vi "SLSC_Example_AsyscRTEnginer.vi"(10 "Parameters":variant, 11 "Process":refnum<class "Process.lvclass">) -> ()   [LabVIEW 2020, in "SLSC EDS Engine.lvlib"]
uses:
  SLSC EDS Engine.lvlib
  <vilib>/NI/NIVS Inline Async API/_VS Inline Async API/Process/Process.lvclass
  Types/Async Engine State Control.ctl
  Shared/Compiled.Settings.ctl
  Shared/SLSC Static Settings.ctl
  SLSC CD API/SLSC CD Engine/SLSC Dynamic Channel.ctl
  SLSC CD API/SLSC CD Engine/SLSC Datatype.ctl
  <vilib>/NI/NIVS Inline Async API/_VS Inline Async API/Process/Process.lvclass/Process.ctl
  <vilib>/NI/NIVS Inline Async API/_Data Access Engine/Access Type Classes/Read/Read.lvclass/Read.ctl
  <vilib>/NI/NIVS Inline Async API/_Data Access Engine/Access Type Classes/ReadWrite/ReadWrite.lvclass/ReadWrite.ctl
  <vilib>/NI/NIVS Inline Async API/_Data Access Engine/Access Type Classes/Write/Write.lvclass/Write.ctl
  <vilib>/NI/NIVS Inline Async API/_Data Access Engine/Data Access Engine/Methods/Read.Data.Detect.vi
  <vilib>/NI/NIVS Inline Async API/_Data Access Engine/Data Access Engine/Methods/Write.Data.vi
  <vilib>/NI/NIVS Inline Async API/_Data Access Engine/Data Access Engine/Methods/ReadWrite.Data.vi
  <vilib>/NI/NIVS Inline Async API/_VS Inline Async API/Process/Data Member Access/Read Data Access.vi
  <vilib>/NI/NIVS Inline Async API/_VS Inline Async API/Error Handling Process/SubVIs/Error.ConvertArray.vi
  <vilib>/NI/NIVS Inline Async API/_Data Access Engine/Access Type Classes/Read/Read.ProcessData.Detect.vi
  <vilib>/NI/NIVS Inline Async API/_Data Access Engine/Access Type Classes/Write/Write.ProcessData.vi
  SLSC CD API/SLSC CD Shared/SLSC Define Resource Name.vi
  <vilib>/NI/NIVS Inline Async API/_Data Access Engine/Access Type Classes/ReadWrite/ReadWrite.ProcessData.vi
  <vilib>/NI/NIVS Inline Async API/_Data Access Engine/Access Type Classes/Write/Write.Buffer.vi
  <vilib>/NI/NIVS Inline Async API/_Data Access Engine/Access Type Classes/Write/Write.Commit.vi
  Shared/Constants.vi
  <vilib>/SLSC/Initialize Session with Devices.vi
  <vilib>/SLSC/Set Generic Property.vi
  <vilib>/SLSC/Set Generic Property (Bool).vi
  <vilib>/SLSC/Set Generic Property (DBL).vi
  <vilib>/SLSC/Set Generic Property (I32).vi
  <vilib>/SLSC/Set Generic Property (I64).vi
  <vilib>/SLSC/Set Generic Property (String).vi
  <vilib>/SLSC/Set Generic Property (U32).vi
  <vilib>/SLSC/Set Generic Property (U64).vi
  SLSC CD API/SLSC CD Shared/SLSC Error Suppression.vi
  <vilib>/SLSC/Commit Properties.vi
  <vilib>/SLSC/Commit Properties for Devices.vi
  <vilib>/SLSC/Execute Command.vi
  <vilib>/SLSC/Execute Device Command.vi
  <vilib>/SLSC/Execute Phys Chan Command.vi
  <vilib>/SLSC/Get Generic Property.vi
  <vilib>/SLSC/Get Generic Property (Bool).vi
  <vilib>/SLSC/Get Generic Property (DBL).vi
  <vilib>/SLSC/Get Generic Property (I32).vi
  <vilib>/SLSC/Get Generic Property (I64).vi
  <vilib>/SLSC/Get Generic Property (String).vi
  <vilib>/SLSC/Get Generic Property (U32).vi
  <vilib>/SLSC/Get Generic Property (U64).vi
  <vilib>/SLSC/Close Session.vi
  <vilib>/NI/NIVS Inline Async API/_Data Access Engine/Data Access Engine/Data Access Engine.lvclass
  <vilib>/NI/NIVS Inline Async API/_Data Access Engine/Data Access Engine/Methods/ReadWrite.Lookup.vi
  <vilib>/NI/NIVS Inline Async API/_Data Access Engine/Data Access Engine/Methods/Write.Lookup.vi
  <vilib>/NI/NIVS Inline Async API/_Data Access Engine/Data Access Engine/Methods/Read.Lookup.vi
  <vilib>/SLSC/SLSC.lvlib
  Shared/SLSC EDS Shared.lvlib
  SLSC CD API/SLSC CD Shared/SLSC CD Shared.lvlib
  SLSC CD API/SLSC CD Engine/SLSC CD Engine.lvlib
  <vilib>/NI VeriStand/Custom Device Tools/Custom Device Utility Library/Custom Device Utility Library.lvlib
  <vilib>/NI/NIVS Inline Async API/_Data Access Engine/Access Type Classes/Write/Write.lvclass
panel:
  out "LoopRate(ms)":u32=50
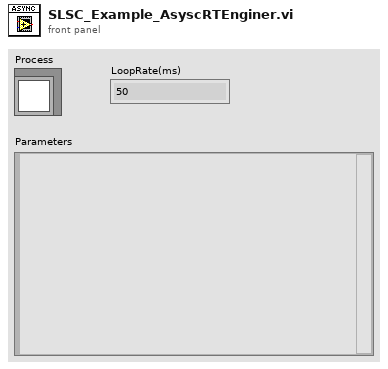
[diagram p1: front panel]
types:
  T1 = typedef "SLSC EDS Engine.lvlib/Async Engine State Control.ctl" = enum16{"Initialize", "Configure", "Run", "Reset", "Shutdown"}
  T2 = typedef "SLSC EDS Shared.lvlib/Compiled.Settings.ctl" = cluster{"Name":string, "SLSC Name or IP Address":string, "Slot #":i32, "Reservation Access":i32, "Reservation Group":string, "Configuration Data":T3, "SLSC Get/Read Properties":T4[], "SLSC Set/Write Properties":T4[], "SLSC Dynamic Commands":T4[], "Support Modules":cluster{"Dev.ProductNumber":u32, "Dev.VendorNumber":u32}[]}
  T3 = typedef "SLSC EDS Shared.lvlib/SLSC Static Settings.ctl" = cluster{"Properties":cluster{"Boolean Properties":cluster{"property":refnum<k21>, "Value":bool, "SLSC Item":refnum<k21>, "reset value":bool}[], "Double Properties":cluster{"property":refnum<k21>, "Double Write":dbl, "SLSC Item":refnum<k21>, "Double Reset Value":dbl}[], "I32 Properties":cluster{"property":refnum<k21>, "Int32 Write":i32, "SLSC Item":refnum<k21>, "Int32 Reset Value":i32}[], "I64 Properties":cluster{"property":refnum<k21>, "Int64 Write":i64, "SLSC Item":refnum<k21>, "Int64 Reset Value":i64}[], "String Properties":cluster{"property":refnum<k21>, "String Write":string, "SLSC Item":refnum<k21>, "String Reset Value":string}[], "U32 Properties":cluster{"property":refnum<k21>, "UInt32 Write":u32, "SLSC Item":refnum<k21>, "UInt32 Reset Value":u32}[], "U64 Properties":cluster{"property":refnum<k21>, "UInt64 Write":u64, "SLSC Item":refnum<k21>, "UInt64 Reset Value":u64}[]}, "Commands":T4[], "Reset Commands":T4[], "Apply Values on Deployment":bool, "Apply Reset on Undeployment":bool, "Change Commands":T4[]}
  T4 = typedef "SLSC CD Shared.lvlib/SLSC Dynamic Channel.ctl" = cluster{"SLSC Item":string, "property":string, "Data Type":T5}
  T5 = typedef "SLSC CD Shared.lvlib/SLSC Datatype.ctl" = enum16{"Bool", "Double", "I32", "I64", "String", "U32", "U64"}
  T6 = typedef "Data Access Engine.lvlib/Data Access Engine.lvclass/Write.DVR.ctl" = refnum<data-value>
  T7 = typedef "Data Access Engine.lvlib/Data Access Engine.lvclass/Read.DVR.ctl" = refnum<data-value>
  T8 = typedef "Data Access Engine.lvlib/Data Access Engine.lvclass/ReadWrite.DVR.ctl" = refnum<data-value>
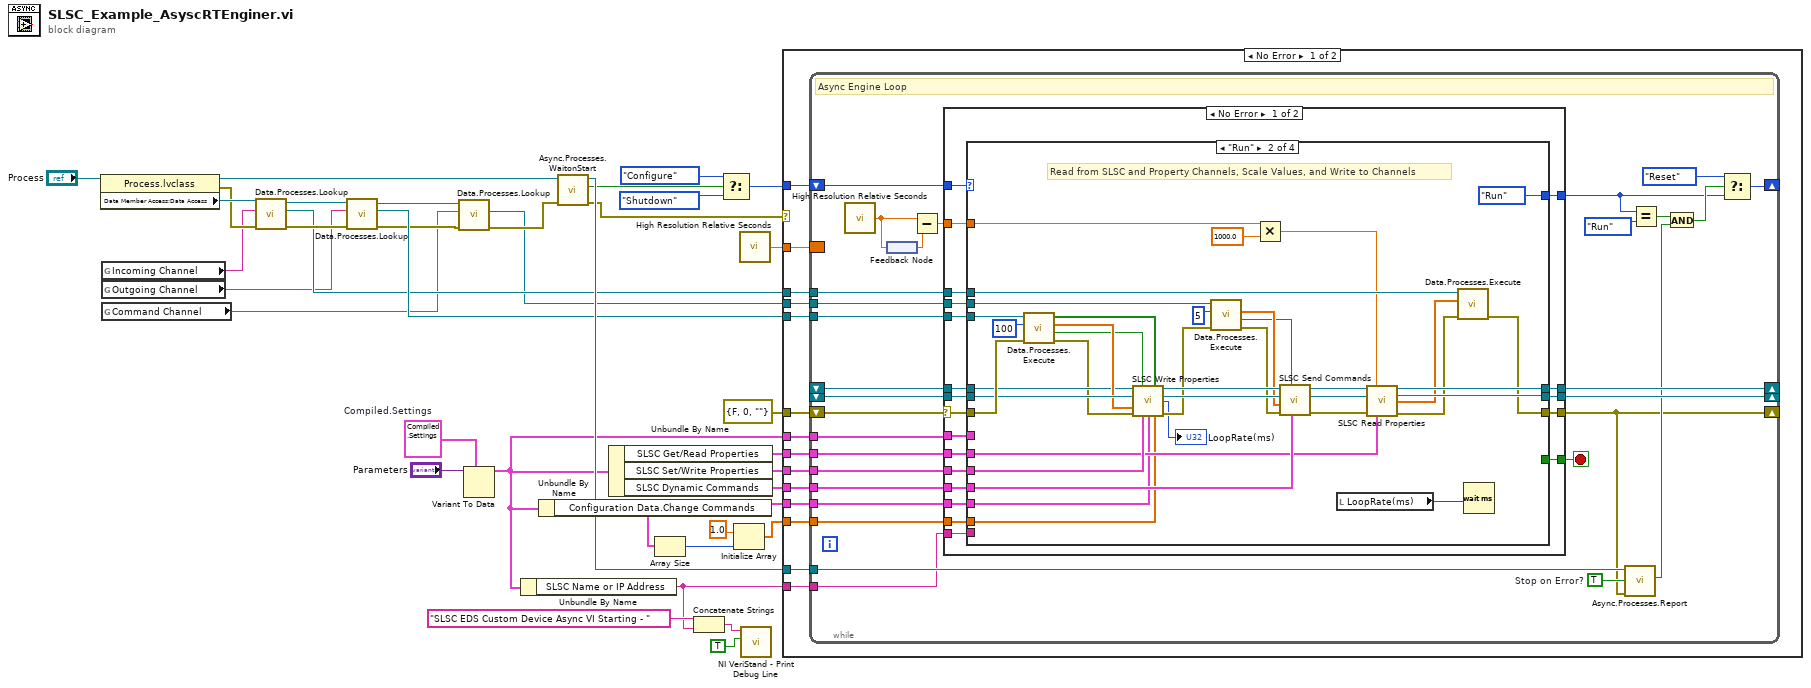
[diagram p0: block diagram]
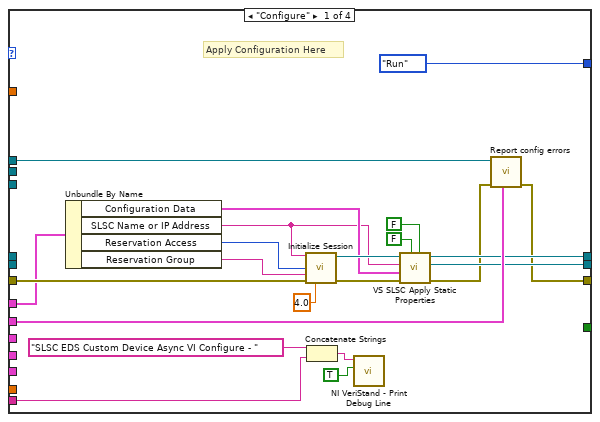
[diagram p2: hidden frame]
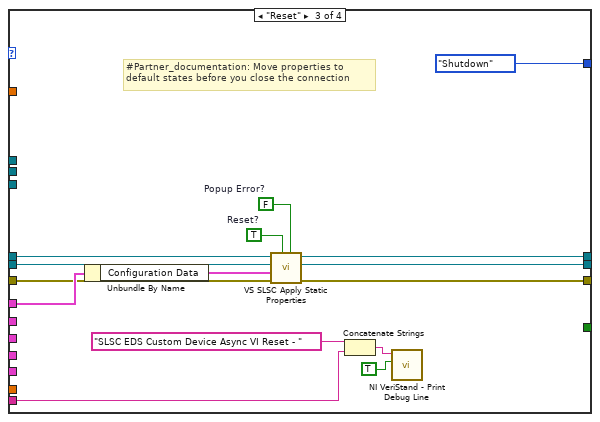
[diagram p3: hidden frame]
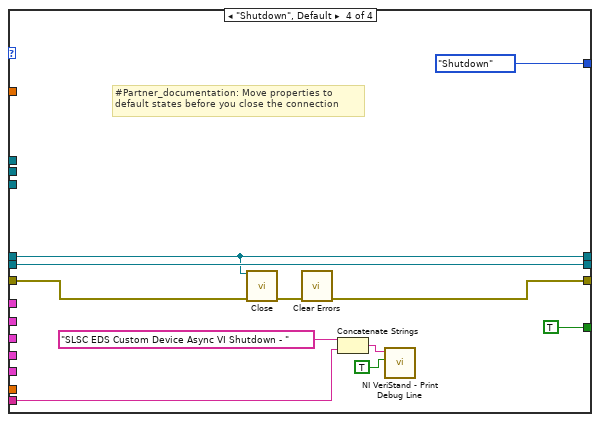
[diagram p4: hidden frame]
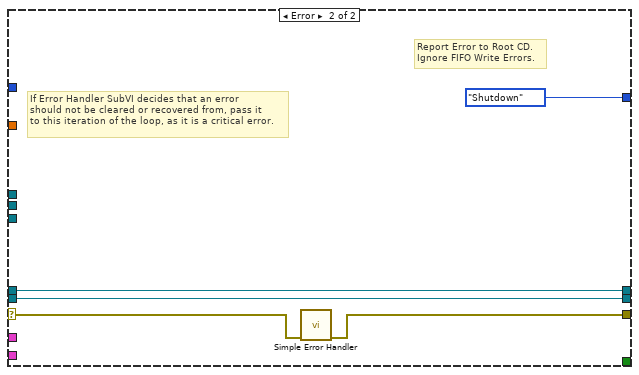
[diagram p5: hidden frame]
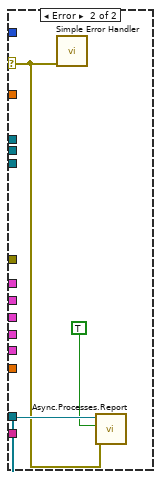
[diagram p6: hidden frame]
diagram:
  w26 = T2 {"Name"="", "SLSC Name or IP Address"="", "Slot #"=0, "Reservation Access"=3, "Reservation Group"="", "Configuration Data"={"Properties"={"Boolean Properties"=[], "Double Properties"=[], "I32 Properties"=[], "I64 Properties"=[], "String Properties"=[], "U32 Properties"=[], "U64 Properties"=[]}, "Commands"=[], "Reset Commands"=[], "Apply Values on Deployment"=TRUE, "Apply Reset on Undeployment"=TRUE, "Change Commands"=[]}, "SLSC Get/Read Properties"=[], "SLSC Set/Write Properties"=[], "SLSC Dynamic Commands"=[], "Support Modules"=[]}  # Compiled.Settings
  n1 = property class="Process.lvclass"(reference="Process") -> (reference out=w30:refnum<class "Process.lvclass">, error out=w28:errorcluster, "Data Member Access:Data Access"=w29:refnum<class "Data Access Engine.lvclass">)  [unwired: 1 in]
  n2 = global read "Constants.vi" "Incoming Channel"() -> (w18:string)
  n3 = global read "Constants.vi" "Outgoing Channel"() -> (w17:string)
  n4 = global read "Constants.vi" "Command Channel"() -> (w12:string)
  n5 = call-poly <vilib>:"Data.Processes.Lookup.vi"("error in (no error)"=w28, "Name"=w18, "Data Access API in"=w29) -> ("error out"=w34:errorcluster, "Ref"=w33:T6, "Data Access API out"=w32:refnum<class "Data Access Engine.lvclass">)  [unwired: 5 in, 1 out]
  n6 = call-poly <vilib>:"Data.Processes.Lookup.vi"("error in (no error)"=w34, "Name"=w17, "Data Access API in"=w32) -> ("error out"=w14:errorcluster, "Ref"=w35:T7, "Data Access API out"=w15:refnum<class "Data Access Engine.lvclass">)  [unwired: 5 in, 1 out]
  n7 = call-poly <vilib>:"Data.Processes.Lookup.vi"("error in (no error)"=w14, "Name"=w12, "Data Access API in"=w15) -> ("error out"=w13:errorcluster, "Ref"=w11:T8)  [unwired: 5 in, 2 out]
  n8 = Variant To Data(type=w26, Variant="Parameters") -> (data=w2:T2)  [unwired: 1 in, 1 out]
  n9 = Unbundle By Name(w2) -> ("SLSC Name or IP Address"=w1:string)
  n10 = Unbundle By Name(w2) -> ("Configuration Data.Change Commands"=w9:T4[])
  n11 = call <vilib>:"Async.Processes.WaitonStart.vi"("error in (no error)"=w13, "Process"=w30) -> ("error out"=w36:errorcluster, "Execute"=w24:bool, "Process out"=w37:refnum<class "Process.lvclass">)  [unwired: 7 in]
  n12 = Unbundle By Name(w2) -> ("SLSC Get/Read Properties"=w20:T4[], "SLSC Set/Write Properties"=w19:T4[], "SLSC Dynamic Commands"=w16:T4[])
  n13 = Array Size(array=w9) -> (size(s)=w7:i32)
  n14 = Concatenate Strings("SLSC EDS Custom Device Async VI Starting - " ("Message"), w1) -> (w3:string)
  n15 = Select(t=Async_Engine_State_Control."Configure", s=w24, f=Async_Engine_State_Control."Shutdown") -> (s? t:f=w21:T1)
  n16 = Initialize Array(1.0 ("element"), w7) -> (w6:dbl[])
  n17 = call <vilib>:"High Resolution Relative Seconds.vi"() -> ("relative seconds"=w10:dbl)
  n18 = call <vilib>:"NI VeriStand - Print Debug Line.vi"("Add to log file? (F)"=TRUE ("Add to log file? (T)"), "Message"=w3) -> ()  [unwired: 9 in, 1 out]
  n19 = case shown="No Error" w36 {
    selector: w36 -> [_ w193]
    tunnel: w37 -> [w51 w194]
    tunnel: w33 -> [w50 _]
    tunnel: w35 -> [w49 _]
    tunnel: w2 -> [w44 _]
    tunnel: errorcluster {"status"=FALSE, "code"=0, "source"=""} ("error IO") -> [w41 _]
    tunnel: w21 -> [w48 _]
    tunnel: w20 -> [w47 _]
    tunnel: w19 -> [w46 _]
    tunnel: w10 -> [w45 _]
    tunnel: w16 -> [w43 _]
    tunnel: w11 -> [w42 _]
    tunnel: w9 -> [w40 _]
    tunnel: w6 -> [w39 _]
    tunnel: w1 -> [w38 _]
    frame No Error {
      n20 = while {
        shift-right: [w56] -> _
        shift-left: w41 -> [w81]
        shift-right: [w64] -> _
        shift-left: w48 -> [w80]
        shift-right: [w78] -> _
        shift-left: _ -> [w77]
        tunnel: w49 -> [w76]
        tunnel: w50 -> [w75]
        tunnel: w51 -> [w74]
        tunnel: w47 -> [w73]
        tunnel: w46 -> [w72]
        shift-right: [w71] -> _
        shift-left: _ -> [w70]
        border: w45 -> [_]
        tunnel: w43 -> [w63]
        tunnel: w42 -> [w62]
        tunnel: w44 -> [w79]
        tunnel: w40 -> [w54]
        tunnel: w39 -> [w53]
        tunnel: w38 -> [w52]
        stop <- w66 stop-if-true
        w69 = TRUE  # Stop on Error?
        # "Async Engine Loop"
        n21 = call <vilib>:"High Resolution Relative Seconds.vi"() -> ("relative seconds"=w55:dbl)
        n22 = feedback-in #1(w55) -> ()
        n23 = feedback #1() -> (w68:dbl)
        n24 = Subtract(x=w55, y=w68) -> (x-y=w67:dbl)
        n25 = case shown="No Error" w81 {
          selector: w81 -> [w100 w188]
          tunnel: [w94 w187] -> w56
          tunnel: w80 -> [w101 _]
          tunnel: [w95 Async_Engine_State_Control."Shutdown"] -> w60
          tunnel: [w99 _] -> w66
          tunnel: w79 -> [w98 _]
          tunnel: [w97 w191] -> w78
          tunnel: w77 -> [w96 w191]
          tunnel: w76 -> [w93 _]
          tunnel: w75 -> [w92 _]
          tunnel: w73 -> [w91 _]
          tunnel: w72 -> [w90 _]
          tunnel: [w89 w189] -> w71
          tunnel: w70 -> [w88 w189]
          tunnel: w67 -> [w87 _]
          tunnel: w63 -> [w86 _]
          tunnel: w62 -> [w85 _]
          tunnel: w54 -> [w84 _]
          tunnel: w53 -> [w83 _]
          tunnel: w52 -> [w82 _]
          frame No Error {
            n26 = case shown="\"Run\"" w101 {
              tunnel: w100 -> [w123 w158 w173 w181]
              tunnel: [w110 w131 w172 w183] -> w94
              tunnel: [Async_Engine_State_Control."Run" Async_Engine_State_Control."Run" Async_Engine_State_Control."Shutdown" Async_Engine_State_Control."Shutdown"] -> w95
              tunnel: [_ _ _ TRUE] -> w99
              tunnel: w98 -> [w121 _ w174 _]
              tunnel: [w118 w151 w166 w182] -> w97
              tunnel: w96 -> [_ w156 w168 w182]
              tunnel: w93 -> [_ w159 _ _]
              tunnel: w92 -> [w120 w135 _ _]
              tunnel: w91 -> [w119 w134 _ _]
              tunnel: w90 -> [_ w154 _ _]
              tunnel: [w117 w152 w167 w180] -> w89
              tunnel: w88 -> [_ w153 w169 w180]
              tunnel: w87 -> [_ w132 _ _]
              tunnel: w86 -> [_ w141 _ _]
              tunnel: w85 -> [_ w133 _ _]
              tunnel: w84 -> [_ w125 _ _]
              tunnel: w83 -> [_ w124 _ _]
              tunnel: w82 -> [w102 _ w161 w176]
              frame "Configure" {
                # "Apply Configuration Here"
                n27 = Unbundle By Name(w121) -> ("Configuration Data"=w109:T3, "SLSC Name or IP Address"=w103:string, "Reservation Access"=w107:i32, "Reservation Group"=w108:string)
                n28 = call-poly <vilib>:"Initialize Session.vi"("devices"=w103, "reservation access (Read/Write)"=w107, "reservation group"=w108, "error in (no error)"=w123, "connect timeout (60 sec)"=4.0 ("connect timeout (10 sec)")) -> ("session out"=w114:refnum<k21>, "error out"=w113:errorcluster)  [unwired: 9 in]
                n29 = Concatenate Strings("SLSC EDS Custom Device Async VI Configure - " ("Message"), w102) -> (w106:string)
                n30 = call <vilib>:"NI VeriStand - Print Debug Line.vi"("Add to log file? (F)"=TRUE ("Add to log file? (T)"), "Message"=w106) -> ()  [unwired: 9 in, 1 out]
                n31 = call "VS SLSC Apply Static Properties.vi"("Popup Error?"=FALSE, "Reset?"=FALSE, "error in (no error)"=w113, "Configuration Data"=w109, "SLSC Module Name in"=w103, "Refnum in"=w114) -> ("error out"=w111:errorcluster, "SLSC Module Name out"=w118:refnum<k21>, "Refnum out"=w117:refnum<k21>)  [unwired: 3 in]
                n32 = call "Report config errors.vi"("SLSC Dynamic Inputs"=w119, "error in (no error)"=w111, "Data Value Reference in"=w120) -> ("error out"=w110:errorcluster)  [unwired: 8 in]
              }
              frame "Run" {
                # "Read from SLSC and Property Channels, Scale Values, and Write to Channels"
                n33 = call-poly <vilib>:"Data.Processes.Execute.vi"("error in (no error)"=w158, "timeout ms"=100, "Ref"=w159) -> ("error out"=w140:errorcluster, "Timeout?"=w137:bool, "Values"=w155:dbl[], "Detect?"=w126:bool[])  [unwired: 5 in]
                n34 = call "SLSC Write Properties.vi"("session in"=w153, "Stop Updating?"=w137, "Detect?"=w126, "SLSC Module Name"=w156, "Values"=w155, "error in"=w140, "SLSC Dynamic Outputs"=w154, "Change Commands"=w125, "Command Values"=w124) -> ("session out"=w147:refnum<k21>, "SLSC Module Name"=w146:refnum<k21>, "LoopRate(ms)"=→"LoopRate(ms)":u32, "error out"=w139:errorcluster)  [unwired: 3 in]
                n35 = call-poly <vilib>:"Data.Processes.Execute.vi"("error in (no error)"=w139, "timeout ms"=5, "Ref"=w133) -> ("error out"=w138:errorcluster, "Timeout?"=w136:bool, "Data"=w143:dbl[])  [unwired: 5 in, 1 out]
                n36 = Multiply(x=w132, y=1000.0) -> (x*y=w130:dbl)
                n37 = call "SLSC Send Commands.vi"("SLSC Dynamic Commands"=w141, "Timeout?"=w136, "error in"=w138, "Values"=w143, "SLSC Module Name"=w146, "session in"=w147) -> ("error out"=w142:errorcluster, "SLSC Module Name"=w144:refnum<k21>, "session out"=w145:refnum<k21>)  [unwired: 3 in]
                n38 = local read "LoopRate(ms)"() -> (w127:u32)
                n39 = call "SLSC Read Properties.vi"("session in"=w145, "LoopDuration(ms)"=w130, "SLSC Module Name"=w144, "error in"=w142, "SLSC Dynamic Inputs"=w134) -> ("session out"=w152:refnum<k21>, "SLSC Module Name"=w151:refnum<k21>, "Values"=w149:dbl[], "error out"=w150:errorcluster)  [unwired: 7 in]
                n40 = call-poly <vilib>:"Data.Processes.Execute.vi"("error in (no error)"=w150, "Values"=w149, "Ref"=w135) -> ("error out"=w131:errorcluster)  [unwired: 8 in]
                n41 = Wait (ms)(milliseconds to wait=w127) -> ()  [unwired: 1 out]
              }
              frame "Reset" {
                w165 = FALSE  # Popup Error?
                w170 = TRUE  # Reset?
                # "#Partner_documentation: Move properties to \ndefault states before you close the connection"
                n42 = Unbundle By Name(w174) -> ("Configuration Data"=w171:T3)
                n43 = call "VS SLSC Apply Static Properties.vi"("Popup Error?"=w165, "Reset?"=w170, "error in (no error)"=w173, "Configuration Data"=w171, "SLSC Module Name in"=w168, "Refnum in"=w169) -> ("error out"=w172:errorcluster, "SLSC Module Name out"=w166:refnum<k21>, "Refnum out"=w167:refnum<k21>)  [unwired: 3 in]
                n44 = Concatenate Strings("SLSC EDS Custom Device Async VI Reset - " ("Message"), w161) -> (w164:string)
                n45 = call <vilib>:"NI VeriStand - Print Debug Line.vi"("Add to log file? (F)"=TRUE ("Add to log file? (T)"), "Message"=w164) -> ()  [unwired: 9 in, 1 out]
              }
              frame "Shutdown", Default {
                # "#Partner_documentation: Move properties to \ndefault states before you close the connection"
                n46 = call-poly <vilib>:"Close.vi"("session in"=w180, "error in (no error)"=w181) -> ("error out"=w184:errorcluster)  [unwired: 13 in]
                n47 = call <vilib>:"Clear Errors.vi"("error in (no error)"=w184) -> ("error out"=w183:errorcluster)  [unwired: 5 in, 1 out]
                n48 = Concatenate Strings("SLSC EDS Custom Device Async VI Shutdown - " ("Message"), w176) -> (w179:string)
                n49 = call <vilib>:"NI VeriStand - Print Debug Line.vi"("Add to log file? (F)"=TRUE ("Add to log file? (T)"), "Message"=w179) -> ()  [unwired: 9 in, 1 out]
              }
            }
          }
          frame Error {
            # "If Error Handler SubVI decides that an error\nshould not be cleared or recovered from, pass it\nto this iteration of the loop, as it is a critical error."
            # "Report Error to Root CD.\nIgnore FIFO Write Errors."
            n50 = call <vilib>:"Simple Error Handler.vi"("error in (no error)"=w188) -> ("error out"=w187:errorcluster)  [unwired: 4 in, 4 out]
          }
        }
        n51 = call <vilib>:"Async.Processes.Report.vi"("Error"=w56, "Stop Async on Error?"=w69, "Process in"=w74) -> ("Stop"=w65:bool)  [unwired: 7 in, 1 out]
        n52 = Equal?(x=w60, y=Async_Engine_State_Control."Run") -> (x = y?=w59:bool)
        n53 = And(x=w59, y=w65) -> (x .and. y?=w61:bool)
        n54 = Select(t=Async_Engine_State_Control."Reset", s=w61, f=w60) -> (s? t:f=w64:T1)
      }
    }
    frame Error {
      n55 = call <vilib>:"Simple Error Handler.vi"("error in (no error)"=w193) -> ()  [unwired: 4 in, 5 out]
      n56 = call <vilib>:"Async.Processes.Report.vi"("Error"=w193, "Stop Async on Error?"=TRUE ("Stop on Error?"), "Process in"=w194) -> ()  [unwired: 7 in, 2 out]
    }
  }
